vi "Parse Channels.vi"(4 "tx channel handle array":u32[](array[numeric]), 5 "ScheduledSDI":bool, 6 "rx channel handle array":u32[](array[numeric]), 7 "FIFO Idx Qs":T1, 8 "error in (no error)":errorcluster, 9 "Access":T3, 10 "Section GUID":string, 11 "Device Reference in":T2 format="%.0x") -> (0 "error out":errorcluster, 1 "Section BaseRate":i32, 2 "Section Data":T4[](array[typedef]) {"Labels Settings"."Label" format="%.0o"}, 3 "Device Reference out":T2 format="%.0x")   [LabVIEW 2015, in "AIT 429 Engine.lvlib"]
uses:
  AIT 429 Engine.lvlib
  RT Controls/RT HW Channel.ctl
  RT Controls/RT Label Settings.ctl
  Shared/Controls and Global/Label.ctl
  Shared/Controls and Global/transferPeriod.ctl
  RT Controls/Driver Data.ctl
  RT Controls/RT Word Settings.ctl
  <vilib>/NI Veristand/Custom Device API/Block Data Reference.ctl
  <vilib>/NI Veristand/Custom Device API/Data Reference.ctl
  RT Controls/RT Param Setting.ctl
  Shared/Controls and Global/Start Bit.ctl
  Shared/Controls and Global/Number of Bits.ctl
  Shared/Controls and Global/TransferType.ctl
  <vilib>/NI Veristand/Custom Device API/Data Access Type.ctl
  <vilib>/NI Veristand/Custom Device API/Custom Device Item Ref.ctl
  RT Controls/FIFO Idx Qs.ctl
  <vilib>/NI Veristand/Custom Device API/Get Item Property (Double).vi
  <vilib>/NI Veristand/Custom Device Tools/Custom Device Utility Library/NI VeriStand - Search for Item by GUID.vi
  Shared/Controls and Global/Global.vi
  <instrlib>/AIT 429/Public/Tx/Data/AIT 429 Set Scheduled Label Transfer Period.vi
  <vilib>/NI Veristand/Custom Device API/Get Item Property (U32).vi
  <vilib>/NI Veristand/Custom Device API/Get Item Property (U16).vi
  <vilib>/NI Veristand/Custom Device Tools/Custom Device Utility Library/Custom Device Utility Library.lvlib
  <vilib>/NI Veristand/Custom Device API/Custom Device API.lvlib
  Shared/AIT 429 Shared.lvlib
  <userlib>/ARINC-429/Owl429.lvlib
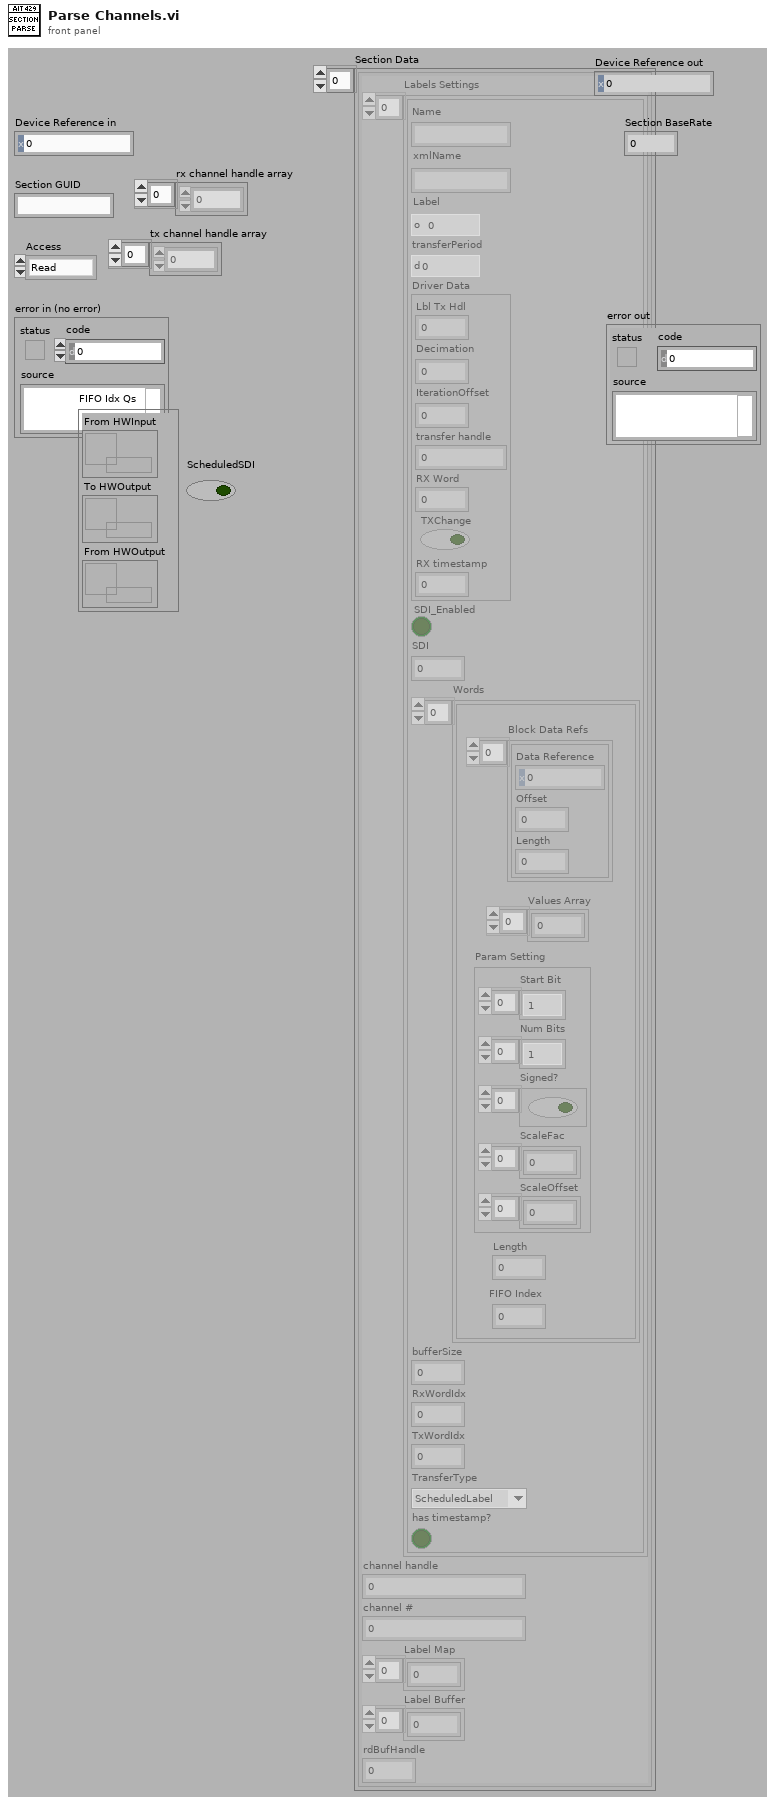
[diagram p1: front panel]
types:
  T1 = typedef "AIT 429 Engine.lvlib/FIFO Idx Qs.ctl" = cluster{"From HWInput":refnum<queue>, "To HWOutput":refnum<queue>, "From HWOutput":refnum<queue>}
  T2 = typedef "Custom Device API.lvlib/Custom Device Item Ref.ctl" = u64
  T3 = typedef "Custom Device API.lvlib/Data Access Type.ctl" = enum16{"Read", "Write"}
  T4 = typedef "AIT 429 Engine.lvlib/RT HW Channel.ctl" = cluster{"Labels Settings":T5[], "channel handle":u32, "channel #":u16, "Label Map":i32[], "Label Buffer":u32[], "rdBufHandle":u32}
  T5 = typedef "AIT 429 Engine.lvlib/RT Label Settings.ctl" = cluster{"Name":string, "xmlName":string, "Label":T6, "transferPeriod":T7, "Driver Data":T8, "SDI_Enabled":bool, "SDI":u8, "Words":T9[], "bufferSize":u32, "RxWordIdx":i32, "TxWordIdx":i32, "TransferType":T15, "has timestamp?":bool}
  T6 = typedef "AIT 429 Shared.lvlib/Label.ctl" = u8
  T7 = typedef "AIT 429 Shared.lvlib/transferPeriod.ctl" = u32
  T8 = typedef "AIT 429 Engine.lvlib/Driver Data.ctl" = cluster{"Lbl Tx Hdl":u32, "Decimation":i32, "IterationOffset":i32, "transfer handle":u32, "RX Word":u32, "TXChange":bool, "RX timestamp":dbl}
  T9 = typedef "AIT 429 Engine.lvlib/RT Word Settings.ctl" = cluster{"Block Data Refs":T10[], "Values Array":dbl[], "Length":i32, "FIFO Index":i32, "Param Setting":T12}
  T10 = typedef "Custom Device API.lvlib/Block Data Reference.ctl" = cluster{"Data Reference":T11, "Offset":u64, "Length":u64}
  T11 = typedef "Custom Device API.lvlib/Data Reference.ctl" = i32
  T12 = typedef "AIT 429 Engine.lvlib/RT Param Setting.ctl" = cluster{"Start Bit":T13[], "Num Bits":T14[], "Signed?":bool[], "ScaleFac":dbl[], "ScaleOffset":dbl[]}
  T13 = typedef "AIT 429 Shared.lvlib/Start Bit.ctl" = i32
  T14 = typedef "AIT 429 Shared.lvlib/Number of Bits.ctl" = i32
  T15 = typedef "AIT 429 Shared.lvlib/TransferType.ctl" = enum16{"ScheduledLabel", "Acyclic", "Block", "Strobe"}
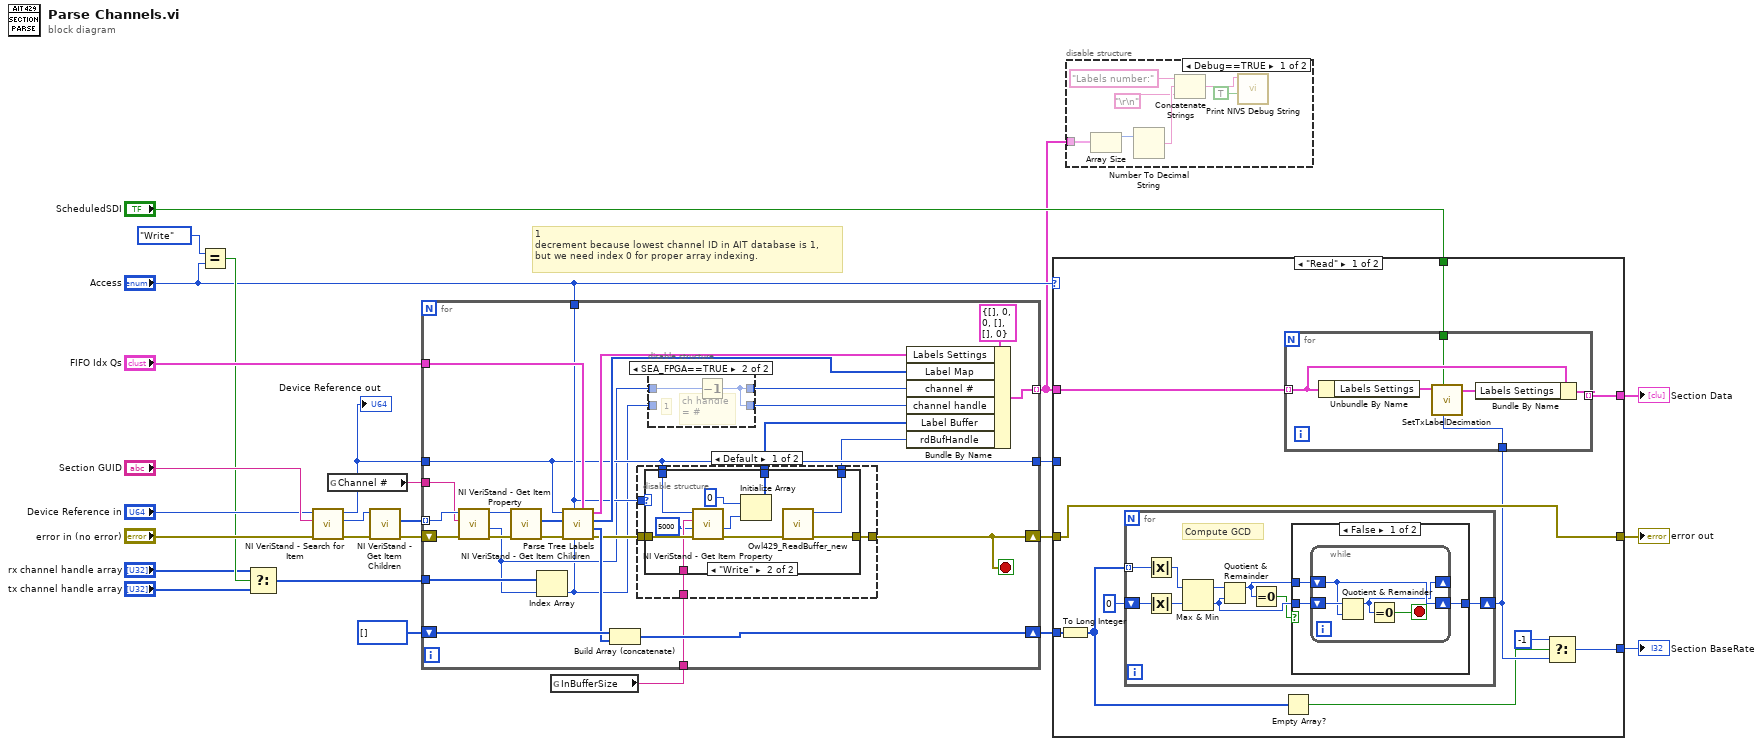
[diagram p0: block diagram]
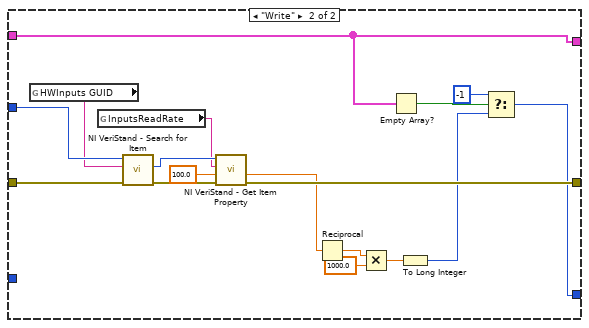
[diagram p4: hidden frame]
diagram:
  # "1\ndecrement because lowest channel ID in AIT database is 1,\nbut we need index 0 for proper array indexing."
  n1 = Equal?(x=Data_Access_Type."Write" ("y"), y="Access") -> (x = y?=w12:bool)
  n2 = Select(t="rx channel handle array", s=w12, f="tx channel handle array") -> (s? t:f=w9:u32[])
  n3 = call-poly <vilib>:"NI VeriStand - Search for Item.vi"("error in"="error in (no error)", "Item GUID"="Section GUID", "Section Ref in"="Device Reference in") -> ("error out"=w21:errorcluster, "Item Ref"=w22:T2, "Section Ref out"=w26:T2)  [unwired: 5 in, 1 out]
  "Device Reference out" <- w26
  n4 = global read "Global.vi" "Channel #"() -> (w4:string)
  n5 = call <vilib>:"NI VeriStand - Get Item Children.vi"("error in (no error)"=w21, "Item Ref in"=w22) -> ("error out"=w25:errorcluster, "Child Refs"=w24:T2[])  [unwired: 6 in, 2 out]
  n6 = global read "Global.vi" "InBufferSize"() -> (w3:string)
  n7 = for {
    tunnel: w24 -> [w44] mode=indexing
    tunnel: "Access" -> [w39]
    tunnel: w26 -> [w37]
    tunnel: [w51] -> w1 mode=indexing
    shift-right: [w33] -> w7
    shift-left: w25 -> [w46]
    shift-right: [w47] -> w17
    shift-left: u32[] [] -> [w49]
    tunnel: w9 -> [w41]
    tunnel: "FIFO Idx Qs" -> [w42]
    tunnel: [w37] -> w5
    tunnel: w4 -> [w36]
    tunnel: w3 -> [w35]
    stop <- w33 stop-if-true
    n8 = call-poly <vilib>:"NI VeriStand - Get Item Property.vi"("error in (no error)"=w46, "Property Name"=w36, "Item Ref in"=w44) -> ("error out"=w45:errorcluster, "Value"=w30:u16, "Item Ref out"=w43:T2)  [unwired: 5 in, 1 out]
    n9 = call <vilib>:"NI VeriStand - Get Item Children.vi"("error in (no error)"=w45, "Item Ref in"=w43) -> ("error out"=w50:errorcluster, "Child Refs"=w31:T2[])  [unwired: 6 in, 2 out]
    n10 = Index Array(array=w41, index=w30) -> (element=w28:u32)
    n11 = call "Parse Tree Labels.vi"("FIFO Idx Qs"=w42, "Channel handle in"=w28, "Access"=w39, "error out"=w50, "Label Refs"=w31, "Custom Device Ref"=w37) -> ("error out"=w38:errorcluster, "Transfer Periods"=w48:u32[], "Label Map"=w40:i32[], "Label data"=w52:T5[])  [unwired: 2 in]
    n12 = Build Array (concatenate)(w49, w48) -> (w47:u32[])
    n13 = disable-structure shown="Default" {
      disable-tunnel: w39 -> [w64 _]
      disable-tunnel: w38 -> [w63 w76]
      disable-tunnel: w37 -> [w62 _]
      disable-tunnel: w35 -> [w61 _]
      disable-tunnel: [w60 _] -> w34
      disable-tunnel: [w59 w76] -> w33
      disable-tunnel: [w58 _] -> w32
      frame condition #0 (active) {
        n14 = case shown="\"Write\"" w64 {
          tunnel: w63 -> [w65 w74]
          tunnel: w62 -> [_ w75]
          tunnel: w61 -> [_ w73]
          tunnel: [w65 w67] -> w59
          tunnel: [_ w69] -> w60
          tunnel: [_ w66] -> w58
          frame "Read", Default {
          }
          frame "Write" {
            n15 = call-poly <vilib>:"NI VeriStand - Get Item Property.vi"("error in (no error)"=w74, "Default Value"=u32 5000, "Property Name"=w73, "Item Ref in"=w75) -> ("error out"=w68:errorcluster, "Value"=w71:u32)  [unwired: 4 in, 2 out]
            n16 = Initialize Array(u32 0 ("element"), w71) -> (w69:u32[])
            n17 = call <userlib>:"Owl429_ReadBuffer_new.vi"("error in (no error)"=w68) -> ("error out"=w67:errorcluster, "buffer handle"=w66:u32)  [unwired: 9 in]
          }
        }
      }
      frame condition #1 {
      }
    }
    n18 = disable-structure shown="SEA_FPGA==TRUE" {
      disable-tunnel: w30 -> [w55 w57]
      disable-tunnel: [w55 w56] -> w29
      disable-tunnel: w28 -> [w54 _]
      disable-tunnel: [w54 w56] -> w27
      frame condition #0 (active) {
      }
      frame condition #1 {
        # "1"
        # "ch handle\n= #"
        n19 = Decrement(x=w57) -> (x-1=w56:u16)
      }
    }
    n20 = Bundle By Name(cluster=T4 {"Labels Settings"=[], "channel handle"=0, "channel #"=0, "Label Map"=[], "Label Buffer"=[], "rdBufHandle"=0} ("HW Channel"), "Labels Settings"=w52, "Label Map"=w40, "channel #"=w29, "channel handle"=w27, "Label Buffer"=w34, "rdBufHandle"=w32) -> (w51:T4)
  }
  n21 = case shown="\"Read\"" "Access" {
    tunnel: w17 -> [w87 _]
    tunnel: w1 -> [w85 w114]
    tunnel: [w81 w111] -> w16
    tunnel: [w84 w114] -> w15
    tunnel: [w83 w121] -> w8
    tunnel: w7 -> [w83 w127]
    tunnel: w5 -> [_ w126]
    tunnel: "ScheduledSDI" -> [w82 _]
    frame "Read" {
      n22 = To Long Integer(number=w87) -> (32bit integer=w80:i32[])
      n23 = for {
        tunnel: w80 -> [w88] mode=indexing
        shift-right: [w90] -> w79
        shift-left: 0 ("gcd(x,y)") -> [w89]
        # "Compute GCD"
        n24 = Absolute Value(x=w88) -> (abs(x)=w95:i32)
        n25 = Absolute Value(x=w89) -> (abs(x)=w96:i32)
        n26 = Max & Min(x=w95, y=w96) -> (max(x,y)=w91:i32, min(x,y)=w93:i32)
        n27 = Quotient & Remainder(x=w91, y=w93) -> (x-y*floor(x/y)=w94:i32)  [unwired: 1 out]
        n28 = Equal To 0?(x=w94) -> (x = 0?=w92:bool)
        n29 = case shown="False" w92 {
          tunnel: [w99 w104] -> w90
          tunnel: w93 -> [w98 w104]
          tunnel: w94 -> [w97 _]
          frame False {
            n30 = while {
              shift-right: [w101] -> w99
              shift-left: w98 -> [w102]
              shift-right: [w100] -> _
              shift-left: w97 -> [w101]
              stop <- w103 stop-if-true
              n31 = Quotient & Remainder(x=w102, y=w101) -> (x-y*floor(x/y)=w100:i32)  [unwired: 1 out]
              n32 = Equal To 0?(x=w100) -> (x = 0?=w103:bool)
            }
          }
          frame True {
          }
        }
      }
      n33 = Empty Array?(array=w80) -> (empty?=w78:bool)
      n34 = for {
        tunnel: w85 -> [w109] mode=indexing
        tunnel: w79 -> [w106]
        tunnel: [w107] -> w84 mode=indexing
        tunnel: w82 -> [w105]
        n35 = Unbundle By Name(w109) -> ("Labels Settings"=w110:T5[])
        n36 = call "SetTxLabelDecimation.vi"("SectionBaseRate"=w106, "ScheduledSDI"=w105, "Labels Settings In"=w110) -> ("Label Settings Out"=w108:T5[])  [unwired: 7 in, 1 out]
        n37 = Bundle By Name(cluster=w109, "Labels Settings"=w108) -> (w107:T4)
      }
      n38 = Select(t=-1, s=w78, f=w79) -> (s? t:f=w81:i32)
    }
    frame "Write" {
      n39 = global read "Global.vi" "HWInputs GUID"() -> (w125:string)
      n40 = global read "Global.vi" "InputsReadRate"() -> (w122:string)
      n41 = call-poly <vilib>:"NI VeriStand - Search for Item.vi"("error in"=w127, "Item GUID"=w125, "Section Ref in"=w126) -> ("error out"=w124:errorcluster, "Item Ref"=w123:T2)  [unwired: 5 in, 2 out]
      n42 = call-poly <vilib>:"NI VeriStand - Get Item Property.vi"("error in (no error)"=w124, "Default Value"=100.0, "Property Name"=w122, "Item Ref in"=w123) -> ("error out"=w121:errorcluster, "Value"=w120:dbl)  [unwired: 4 in, 2 out]
      n43 = Reciprocal(x=w120) -> (1/x=w118:dbl)
      n44 = Multiply(x=w118, y=1000.0) -> (x*y=w116:dbl)
      n45 = Empty Array?(array=w114) -> (empty?=w113:bool)
      n46 = To Long Integer(number=w116) -> (32bit integer=w112:i32)
      n47 = Select(t=-1, s=w113, f=w112) -> (s? t:f=w111:i32)
    }
  }
  "Section Data" <- w15
  "error out" <- w8
  "Section BaseRate" <- w16
  n48 = disable-structure shown="Debug==TRUE" {
    disable-tunnel: w1 -> [w131 _]
    frame condition #0 {
      n49 = Array Size(array=w131) -> (size(s)=w130:i32)
      n50 = Number To Decimal String(number=w130) -> (decimal integer string=w129:string)  [unwired: 1 in]
      n51 = Concatenate Strings("Labels number:", w129, "\r\n") -> (w132:string)
      n52 = call "Print NIVS Debug String.vi"("Add to NIVS Log FIle? (T)"=TRUE, "Debug String"=w132) -> ()  [unwired: 8 in, 1 out]
    }
    frame condition #1 (active) {
    }
  }
